vi "Set_Control_Mode.vi"(8 "error in (no error)":errorcluster, 10 "Control Mode":T1, 11 "Motor in":refnum<class "Motor.lvclass">) -> (0 "error out":errorcluster, 3 "Motor out":refnum<class "Motor.lvclass">)   [LabVIEW 2021, in "Motor.lvclass"]
uses:
  Motor.lvclass
  Type_Defs/Control_Mode.ctl
  Motor.lvclass/Motor.ctl
  AnalogOutput/AnalogOutput.lvclass
  ServoDrive/ServoDrive.lvclass
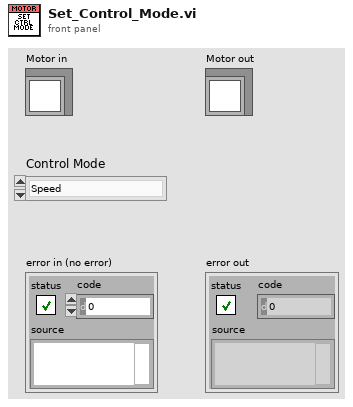
[diagram p1: front panel]
types:
  T1 = typedef "Motor.lvclass/Control_Mode.ctl" = enum16{"Speed", "Torque"}
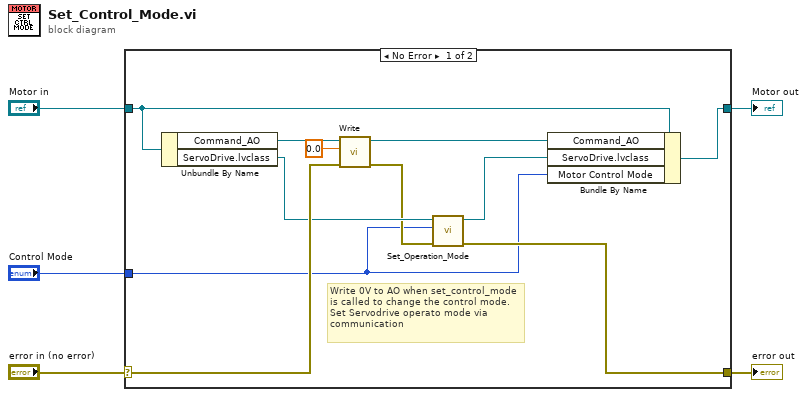
[diagram p0: block diagram]
diagram:
  n1 = case shown="No Error" "error in (no error)" {
    selector: "error in (no error)" -> [w16 w18]
    tunnel: [w8 w18] -> w4
    tunnel: [w15 w17] -> w2
    tunnel: "Motor in" -> [w14 w17]
    tunnel: "Control Mode" -> [w7 _]
    frame No Error {
      # "Write 0V to AO when set_control_mode is called to change the control mode.\nSet Servodrive operato mode via communication"
      n2 = Unbundle By Name(w14) -> ("Command_AO"=w13:refnum<class "AnalogOutput.lvclass">, "ServoDrive.lvclass"=w10:refnum<class "ServoDrive.lvclass">)
      n3 = call-dynamic "Write.vi"("error in (no error)"=w16, "data in"=0.0, "AnalogOutput in"=w13) -> ("error out"=w9:errorcluster, "AnalogOutput out"=w11:refnum<class "AnalogOutput.lvclass">)  [unwired: 7 in]
      n4 = call-dynamic "Set_Operation_Mode.vi"("error in (no error)"=w9, "Motor Control Mode"=w7, "ServoDrive in"=w10) -> ("error out"=w8:errorcluster, "ServoDrive out"=w6:refnum<class "ServoDrive.lvclass">)  [unwired: 7 in]
      n5 = Bundle By Name(cluster=w14, "Command_AO"=w11, "ServoDrive.lvclass"=w6, "Motor Control Mode"=w7) -> (w15:refnum<class "Motor.lvclass">)
    }
    frame Error {
    }
  }
  "error out" <- w4
  "Motor out" <- w2
